vi "Process.vi"(8 "error in":errorcluster, 11 "Plugin in":refnum<class "NVH Condition Indicators.lvclass">) -> (0 "error out":errorcluster, 3 "Plugin out":refnum<class "NVH Condition Indicators.lvclass">)   [LabVIEW 2026, in "NVH Condition Indicators.lvlib" / "NVH Condition Indicators.lvclass"]
uses:
  NVH Condition Indicators.lvclass
  NVH Condition Indicators.lvclass/NVH Condition Indicators.ctl
  <vilib>/FlexLogger/SDK/PluginSDK.lvlibp/PEFClasses/SDK/Plugin/DataHelpers/Write 1D Wfm (DBL)_v2.vi
  <vilib>/FlexLogger/SDK/PluginSDK.lvlibp/PEFClasses/SDK/Plugin/Plugin.lvclass
  Vibration-Core/Calculations.lvlib
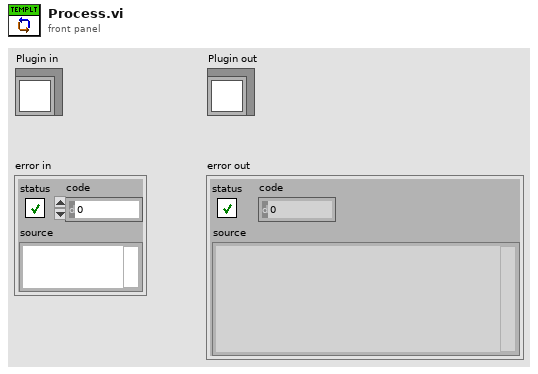
[diagram p1: front panel]
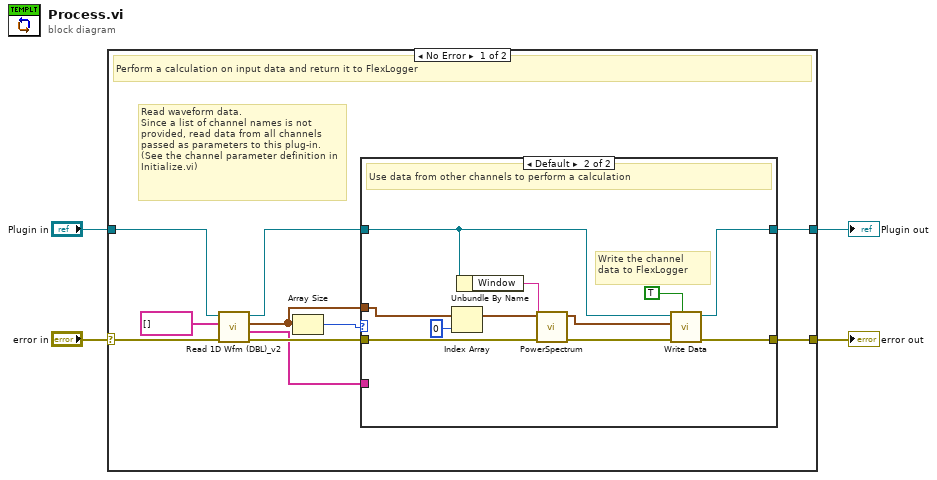
[diagram p0: block diagram]
diagram:
  n1 = case shown="No Error" "error in" {
    selector: "error in" -> [w13 w28]
    tunnel: [w11 w29] -> w1
    tunnel: "Plugin in" -> [w14 w29]
    tunnel: [w12 w28] -> w2
    frame No Error {
      # "Read waveform data.\nSince a list of channel names is not provided, read data from all channels passed as parameters to this plug-in.\n(See the channel parameter definition in Initialize.vi)"
      # "Perform a calculation on input data and return it to FlexLogger"
      n2 = call <vilib>:"Read 1D Wfm (DBL)_v2.vi"("error in (no error)"=w13, "Unique Identifiers (empty = all)"=string[] [] ("Unique Channel Identifers (empty = all)"), "Plugin in"=w14) -> ("error out"=w7:errorcluster, "Stream Names"=w5:string[], "Data"=w10:waveform(dbl)[], "Plugin out"=w8:refnum<class "NVH Condition Indicators.lvclass">)  [unwired: 5 in]
      n3 = Array Size(array=w10) -> (size(s)=w9:i32)
      n4 = case shown="Default" w9 {
        tunnel: w10 -> [_ w25]
        tunnel: [w15 w27] -> w12
        tunnel: [w16 w26] -> w11
        tunnel: w8 -> [w16 w21]
        tunnel: w7 -> [w15 w24]
        tunnel: w5 -> [_ _]
        frame 0 {
          # "No channels sending data to the plugin"
        }
        frame Default {
          # "Write the channel data to FlexLogger"
          # "Use data from other channels to perform a calculation"
          n5 = Index Array(array=w25, index=0) -> (element=w19:waveform(dbl))
          n6 = Unbundle By Name(w21) -> ("Window"=w20:string)
          n7 = call "PowerSpectrum.vi"("error in (no error)"=w24, "Window"=w20, "Data In"=w19) -> ("error out"=w23:errorcluster, "Array of Waveforms"=w22:waveform(dbl)[])  [unwired: 6 in, 1 out]
          n8 = call-poly <vilib>:"Write Data.vi"("Auto Calculate T0 (f)"=TRUE, "error in (no error)"=w23, "Data"=w22, "Plugin in"=w21) -> ("error out"=w27:errorcluster, "Plugin out"=w26:refnum<class "NVH Condition Indicators.lvclass">)  [unwired: 6 in]
        }
      }
    }
    frame Error {
    }
  }
  "error out" <- w2
  "Plugin out" <- w1
